vi "Parse Controls.vi"(8 "error in (no error)":errorcluster, 10 "VI Type":T1(ring), 11 "Controls[]":refnum<vi>[](array[refnum])) -> (0 "error out":errorcluster, 1 "References":refnum<vi>[](array[refnum]), 2 "Control Descriptions":string[](array[string]), 3 "Control Names":string[](array[string]))   [LabVIEW 2016]
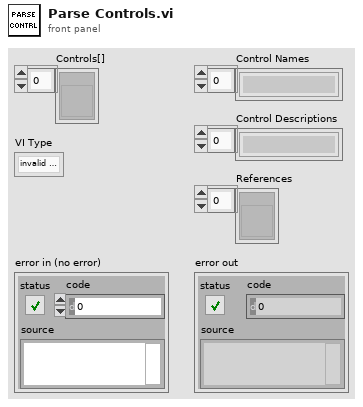
[diagram p1: front panel]
types:
  T1 = enum32{"invalid VI type", "Standard VI", "Control VI", "Global VI", "Polymorphic VI", "Configuration VI", "SubSystem", "Facade VI", "Method VI", "Statechart Diagram VI"}
  T2 = cluster{string, "result string":string, "Description out":string, refnum<vi>}
  T3 = cluster{string, "result string":string, "Description out":string, refnum<vi>}[]
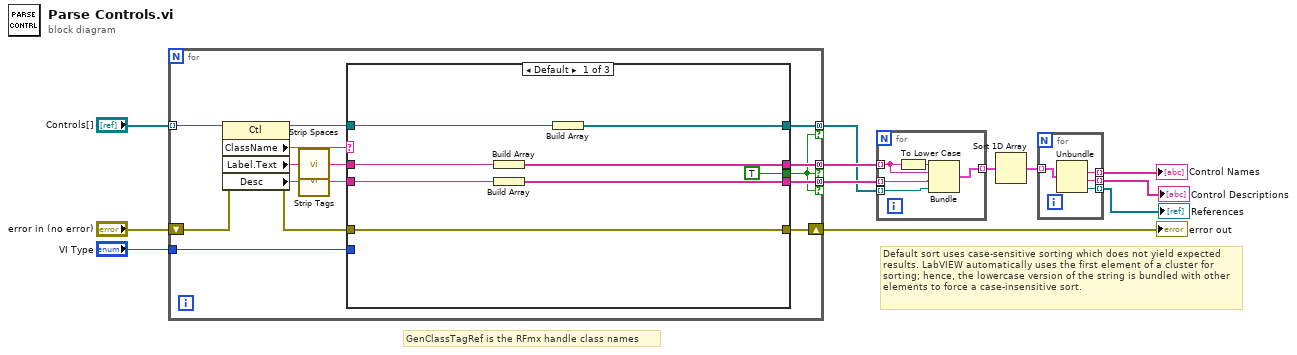
[diagram p0: block diagram]
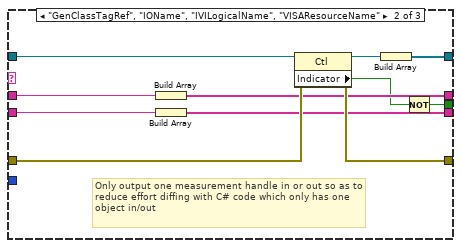
[diagram p2: hidden frame]
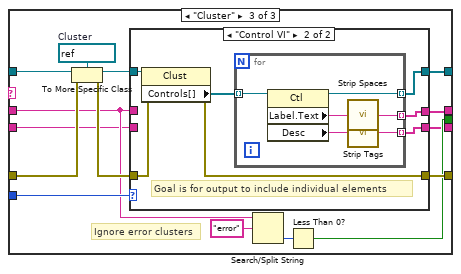
[diagram p3: hidden frame]
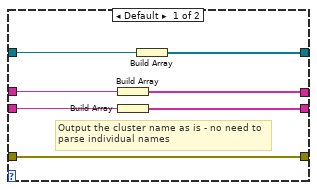
[diagram p4: hidden frame]
diagram:
  # "Default sort uses case-sensitive sorting which does not yield expected results. LabVIEW automatically uses the first element of a cluster for sorting; hence, the lowercase version of the string is bundled with other elements to force a case-insensitive sort."
  # "GenClassTagRef is the RFmx handle class names"
  n1 = for {
    tunnel: "Controls[]" -> [w27] mode=indexing
    shift-right: [w22] -> w10
    shift-left: "error in (no error)" -> [w25]
    tunnel: [w20] -> w8 mode=concatenating if=w13
    tunnel: "VI Type" -> [w19]
    tunnel: [w17] -> w4 mode=concatenating if=w13
    tunnel: [w14] -> w2 mode=concatenating if=w13
    n2 = property class="Ctl"(reference=w27, error in=w25) -> (reference out=w26:refnum<vi>, error out=w23:errorcluster, "ClassName"=w24:string, "Label.Text"=w21:string, "Desc"=w18:string)
    n3 = call "Strip Spaces.vi"("String In"=w21) -> ("result string"=w16:string)  [unwired: 14 in]
    n4 = call "Strip Tags.vi"("Description in"=w18) -> ("Description out"=w15:string)  [unwired: 14 in]
    n5 = case shown="Default" w24 {
      tunnel: w26 -> [w29 w42 w61]
      tunnel: w23 -> [w35 w46 w59]
      tunnel: [w35 w45 w56] -> w22
      tunnel: w16 -> [w32 w43 w50]
      tunnel: [TRUE w40 w53] -> w13
      tunnel: [w33 w44 w52] -> w20
      tunnel: w19 -> [_ _ w51]
      tunnel: w15 -> [w31 w39 w48]
      tunnel: [w30 w38 w49] -> w17
      tunnel: [w28 w36 w47] -> w14
      frame Default {
        n6 = Build Array(w32) -> (w33:string[])
        n7 = Build Array(w31) -> (w30:string[])
        n8 = Build Array(w29) -> (w28:refnum<vi>[])
      }
      frame "GenClassTagRef", "IOName", "IVILogicalName", "VISAResourceName" {
        # "Only output one measurement handle in or out so as to reduce effort diffing with C# code which only has one object in/out"
        n9 = Build Array(w43) -> (w44:string[])
        n10 = Build Array(w39) -> (w38:string[])
        n11 = property class="Ctl"(reference=w42, error in=w46) -> (reference out=w37:refnum<vi>, error out=w45:errorcluster, "Indicator"=w41:bool)
        n12 = Build Array(w37) -> (w36:refnum<vi>[])
        n13 = Not(x=w41) -> (.not. x?=w40:bool)
      }
      frame "Cluster" {
        w58 = refnum<vi> refnum  # Cluster
        # "Ignore error clusters"
        n14 = To More Specific Class(target class=w58, reference=w61, error in=w59) -> (specific class reference=w60:refnum<vi>, error out=w57:errorcluster)
        n15 = case shown="\"Control VI\"" w51 {
          tunnel: w60 -> [w63 w75]
          tunnel: w57 -> [w68 w74]
          tunnel: [w68 w73] -> w56
          tunnel: [w67 w72] -> w52
          tunnel: w50 -> [w66 _]
          tunnel: [w64 w70] -> w49
          tunnel: w48 -> [w65 _]
          tunnel: [w62 w69] -> w47
          frame Default {
            # "Output the cluster name as is - no need to parse individual names"
            n16 = Build Array(w66) -> (w67:string[])
            n17 = Build Array(w65) -> (w64:string[])
            n18 = Build Array(w63) -> (w62:refnum<vi>[])
          }
          frame "Control VI" {
            # "Goal is for output to include individual elements"
            n19 = property class="Clust"(reference=w75, error in=w74) -> (error out=w73:errorcluster, "Controls[]"=w71:refnum<vi>[])  [unwired: 1 out]
            n20 = for {
              tunnel: w71 -> [w81] mode=indexing
              tunnel: [w79] -> w72 mode=indexing
              tunnel: [w77] -> w70 mode=indexing
              tunnel: [w76] -> w69 mode=indexing
              n21 = property class="Ctl"(reference=w81) -> (reference out=w76:refnum<vi>, "Label.Text"=w80:string, "Desc"=w78:string)  [unwired: 1 in, 1 out]
              n22 = call "Strip Spaces.vi"("String In"=w80) -> ("result string"=w79:string)  [unwired: 14 in]
              n23 = call "Strip Tags.vi"("Description in"=w78) -> ("Description out"=w77:string)  [unwired: 14 in]
            }
          }
        }
        n24 = Search/Split String(string=w50, search string/char (-)="error") -> (offset of match=w54:i32)  [unwired: 1 in, 2 out]
        n25 = Less Than 0?(x=w54) -> (x < 0?=w53:bool)
      }
    }
  }
  "error out" <- w10
  n26 = for {
    tunnel: w8 -> [w86] mode=indexing
    tunnel: [w84] -> w7 mode=indexing
    tunnel: w4 -> [w83] mode=indexing
    tunnel: w2 -> [w82] mode=indexing
    n27 = To Lower Case(string=w86) -> (all lower case string=w85:string)
    n28 = Bundle(w85, "result string"=w86, "Description out"=w83, w82) -> (w84:T2)  [unwired: 1 in]
  }
  n29 = Sort 1D Array(array=w7) -> (sorted array=w6:T3)
  n30 = for {
    tunnel: w6 -> [w90] mode=indexing
    tunnel: [w89] -> w5 mode=indexing
    tunnel: [w88] -> w3 mode=indexing
    tunnel: [w87] -> w1 mode=indexing
    n31 = Unbundle(w90) -> ("result string"=w89:string, "Description out"=w88:string, w87:refnum<vi>)  [unwired: 1 out]
  }
  "Control Names" <- w5
  "Control Descriptions" <- w3
  "References" <- w1
